vi "Visu acqui 2.vi"() -> ()   [LabVIEW 2022 SP3]
uses:
  Enum/Enum 7.ctl
  Variables globales/Variable glob generale.vi
  Variables globales/Variable globale compteurs.vi
  Variables globales/Variable glob Keller.vi
  Variables globales/Variable glob Pt.vi
  Variables globales/Variable glob Leybold.vi
  Variables globales/Variable glob Edwards.vi
  Variables globales/Variable glob Th.vi
  Variables globales/Variables glob EUROTHERM.vi
  Variables globales/Variable glob alertes pressions.vi
  Variables globales/Variable glob alertes min-max temperatures.vi
  Variables globales/Variable glob alertes ecart temperatures.vi
  Variables globales/Variable glob alertes Keller.vi
  Variables globales/Variable glob alertes Compteurs.vi
  <vilib>/Utility/config.llb/Write Key (String).vi
  <vilib>/Utility/config.llb/NI_LVConfig.lvlib
panel:
  in  "Légende":T1(array[cluster])
  out "Alerte Compteurs":bool
  in  "voir compteurs":bool caption="Valeurs compteurs"
  in  "Unités par":u16(ring) items=["seconde", "minute", "heure"]
  out "Pente":dbl format="%#.2g"
  in  "Capteur":u16(ring) items=["Puissance Reg REG_TABLE", "Mesure Reg REG_TABLE", "Consigne Reg REG_TABLE", "Sécurité Reg REG_TABLE", "Alarme basse Reg REG_TABLE", "Alarme haute RegREG_TABLE"]
  in  "Calcul Pente":bool
  in  "voir alertes":bool caption="Définitions Alertes"
  out "nb capt":i32
  out "Cuve":string
  out "Dossier distant":path
  out "référence en sortie":refnum<vi>
  out "SORTIE VISU":bool
  in  "Tout Y2":bool
  out "commentaire":string
  out "Dossier de sauvegarde":path
  in  "Tout Y1":bool
  in  "Tout OFF":bool
  out "Chemin du fichier local":path
  out "Alerte écart temp":bool caption="Alerte écarts températures"
  in  "Y2 log":bool caption="Y2 lin"
  in  "Y1 log":bool caption="Y1 lin"
  out "Alerte Keller":bool
  out "Alerte min/max temp":bool caption="Alerte min/max températures"
  out "Alerte vide":bool
  in  "grille Y2":bool
  in  "grille Y1":bool
  out "Courbe":cluster{dbl[], dbl[]}[](graph)
  in  "Echelles des Axes":bool=TRUE
  in  "SORTIR VISU":bool
  # "VISUALISATION ACQUISITIONS\ntempératures et pressions EN COURS"
  # "Ce logiciel et les informations qu'il contient, sont la propriété de l’IAS et ne peuvent être diffusés sans l’autorisation de la Station d’étalonnage"
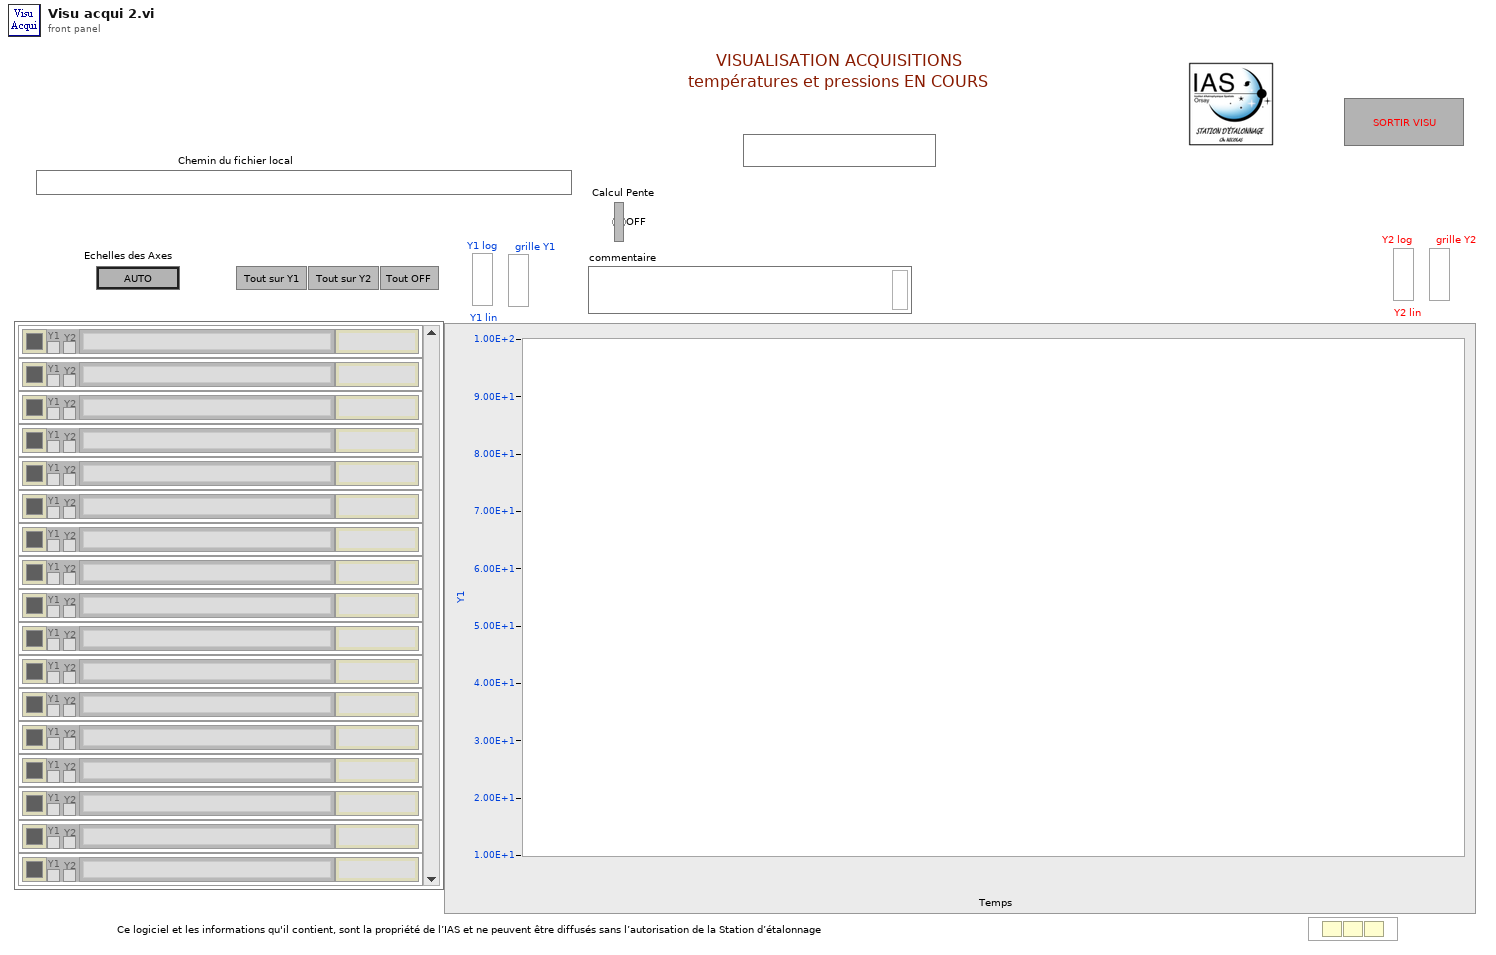
[diagram p1: front panel]
types:
  T1 = cluster{"couleur":u32, "Y1":bool, "nom":string, "donnée":string, "Y2":bool}[]
  T2 = typedef "Enum 7.ctl" = enum16{"init", "choix", "init graph", "visu", "choix 2", "fin"}
  T3 = enum32{"Invalid", "Standard", "Closed", "Hidden", "Minimized", "Maximized"}
  T4 = cluster{"Noms voies select acqui 1COM":string[]}[]
  T5 = cluster{"Nom tache compteurs":refnum<k21>, "Noms des compteurs":string[], "Selection":bool[], "Init compteurs":dbl[], "Noms compteurs selectionnes":string[]}
  T6 = cluster{"Nom tache Pt":refnum<k21>, "Noms des Pt":string[], "Nb Pt":i16, "Selection Pt":bool[], "Nom Pt selectionnees":string[]}[]
  T7 = cluster{"Nom tache Th":refnum<k21>, "Noms des Th":string[], "Nb Th":i16, "Selection Th":bool[], "Nom Th selectionnes":string[]}[]
  T8 = cluster{"couleur":u32, "Y1":bool, "nom":string, "donnée":string, "Y2":bool}
  T9 = cluster{"Alerte temp min/max":bool, "température max":dbl, "température min":dbl, "Défaut min/max temp":bool, "Indices à controler":i16[], "N°":u16}[]
  T10 = cluster{"Indices a controler":i16[], "Defaut":bool, "ecart temp":dbl, "Alerte":bool, ">?":bool, "N°":u16}[]
  T11 = cluster{"Alerte":bool, "valeur alerte":dbl, "Défaut":bool, "Indices à controler":i16[], "N°":u16}[]
  T12 = cluster{"Alerte":bool, "valeur ":dbl, "Défaut":bool, "Indices controler":i16[], "N°":u16}[]
  T13 = cluster{"Alerte Keller":bool, "valeur alerte Keller":dbl, "Défaut Keller":bool, "Indices Keller à controler":i16[], "N°":u16}[]
  T14 = typedef "NI_LVConfig.lvlib/Config Data RefNum.ctl" = refnum<k1>
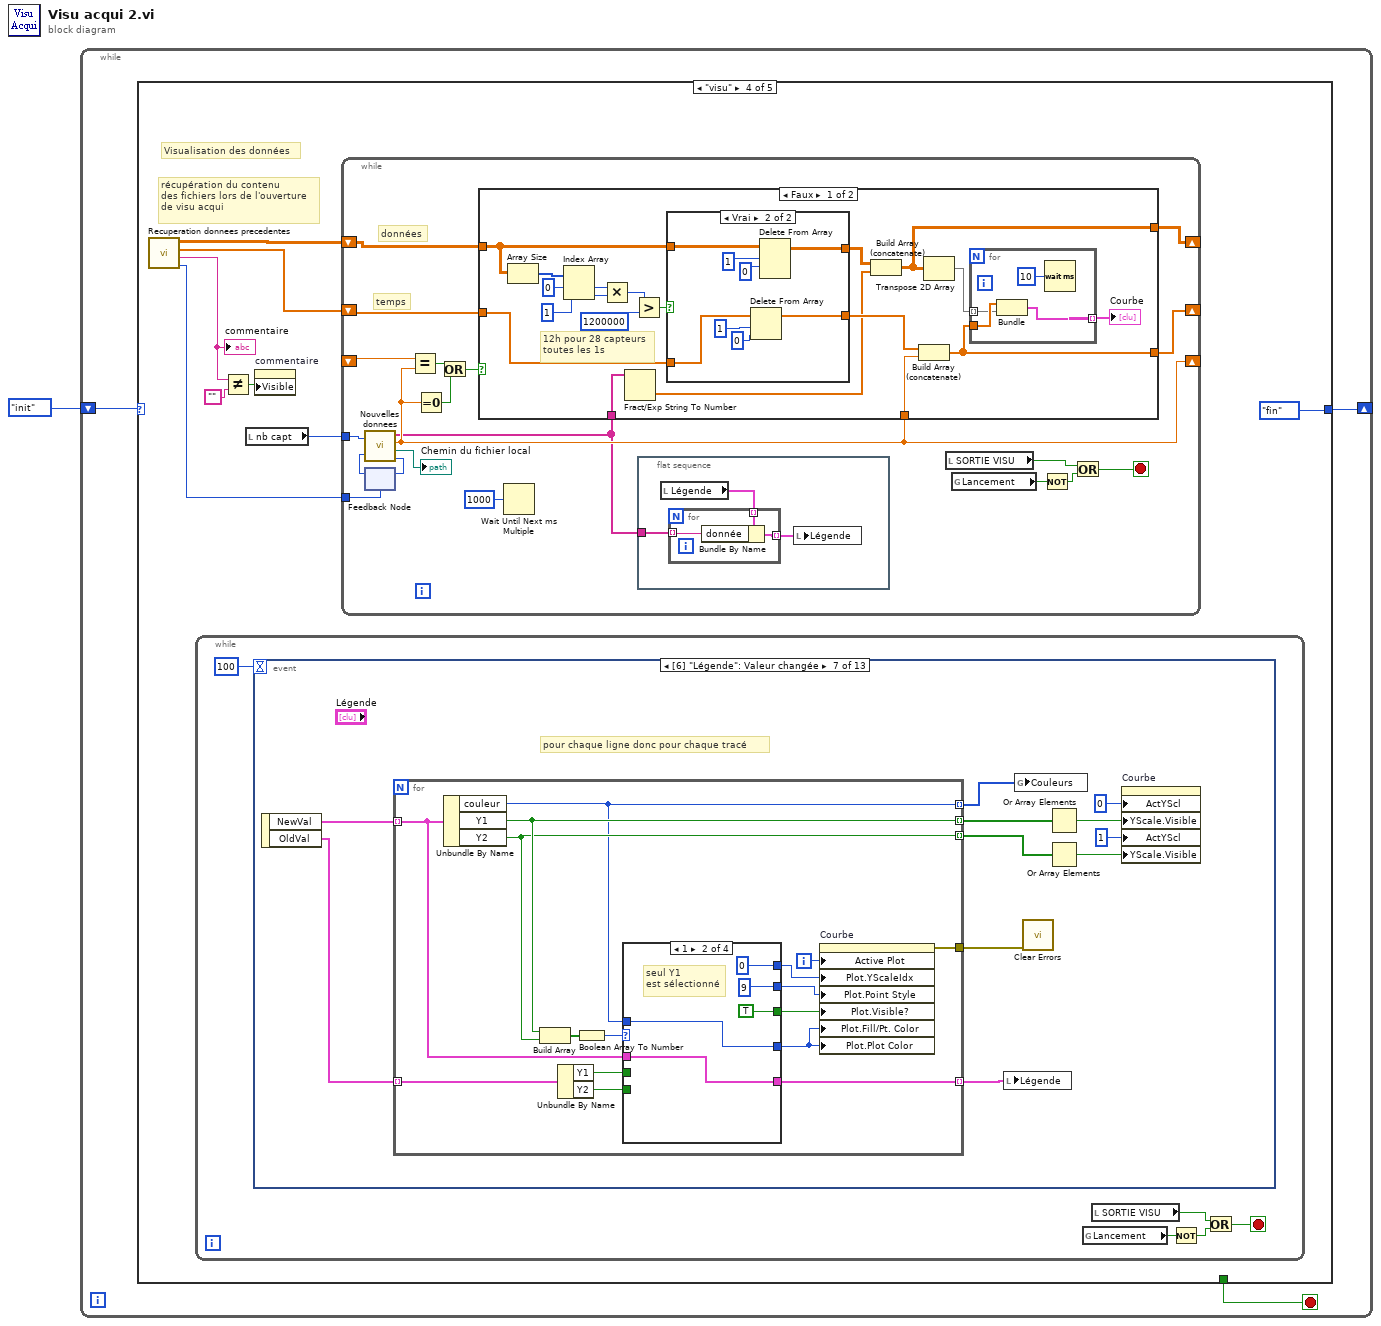
[diagram p0: block diagram]
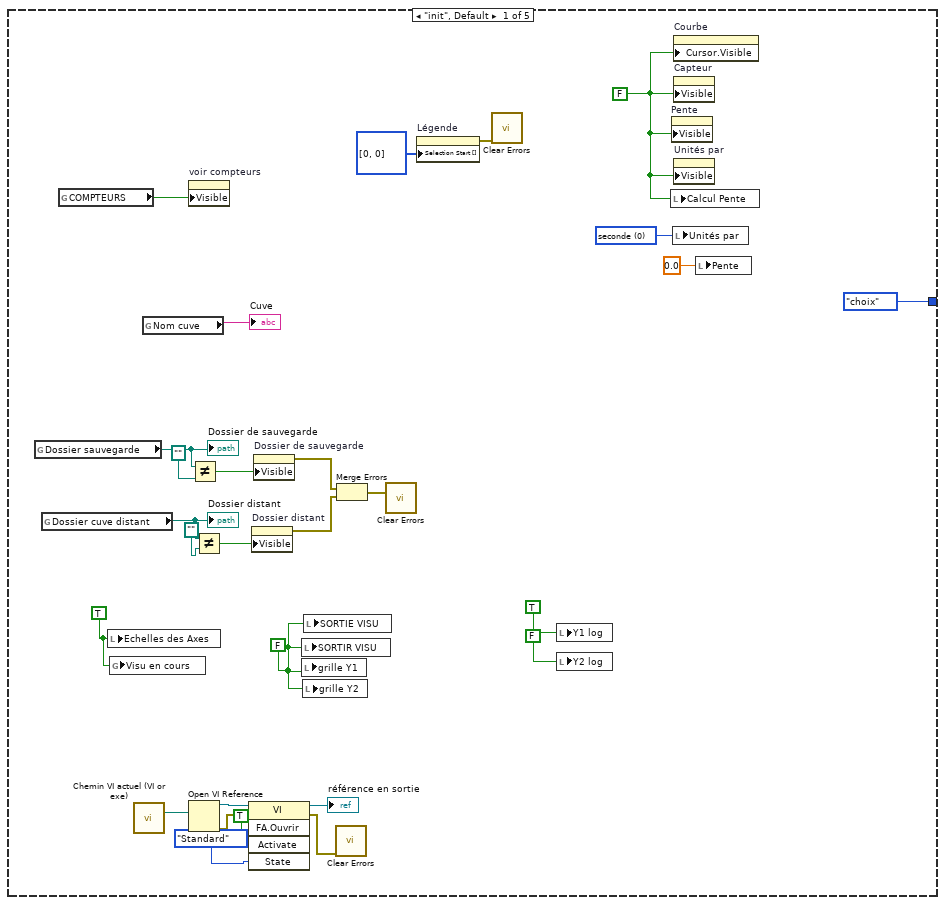
[diagram p2: hidden frame]
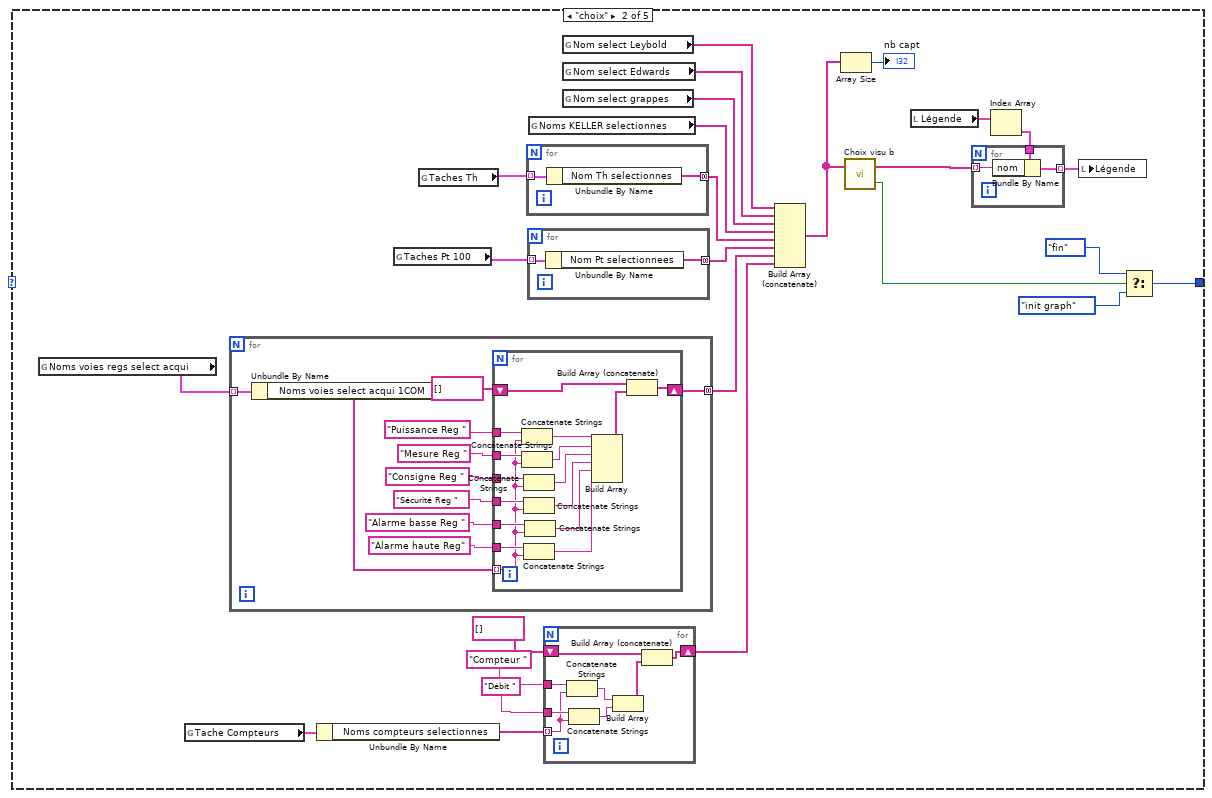
[diagram p3: hidden frame]
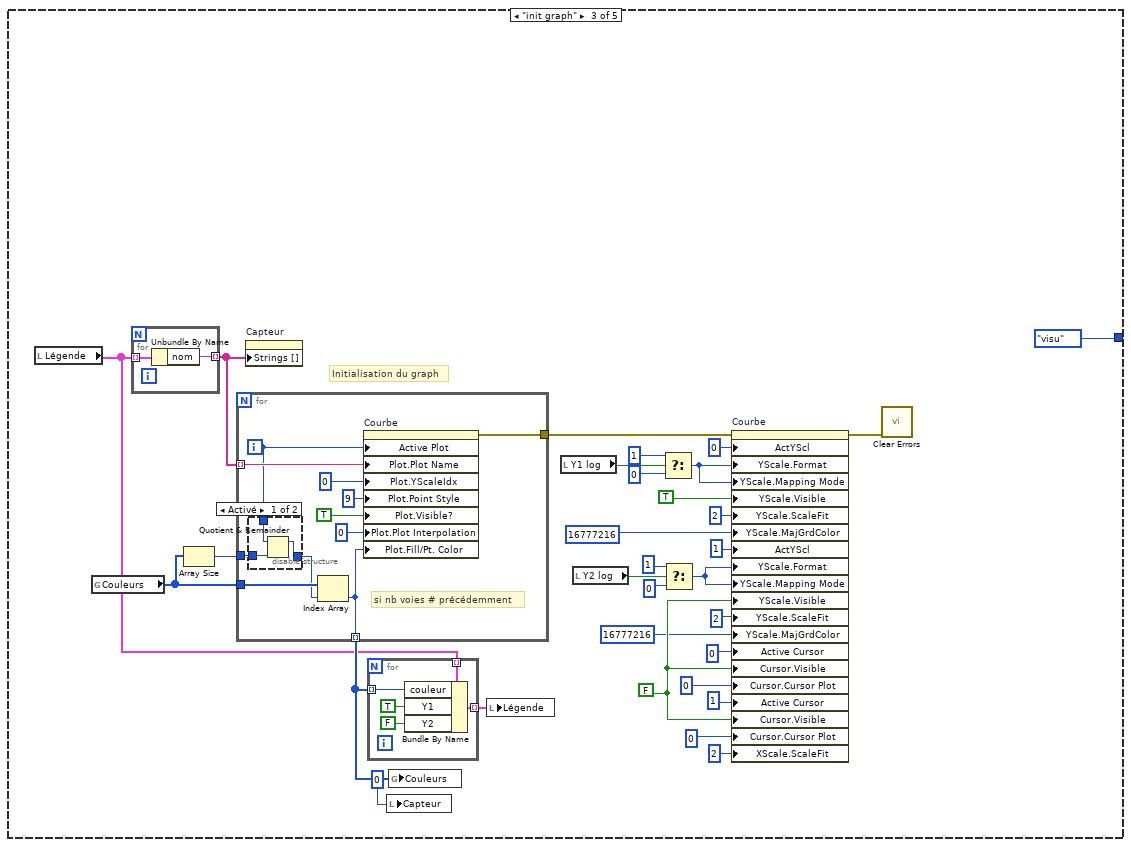
[diagram p4: hidden frame]
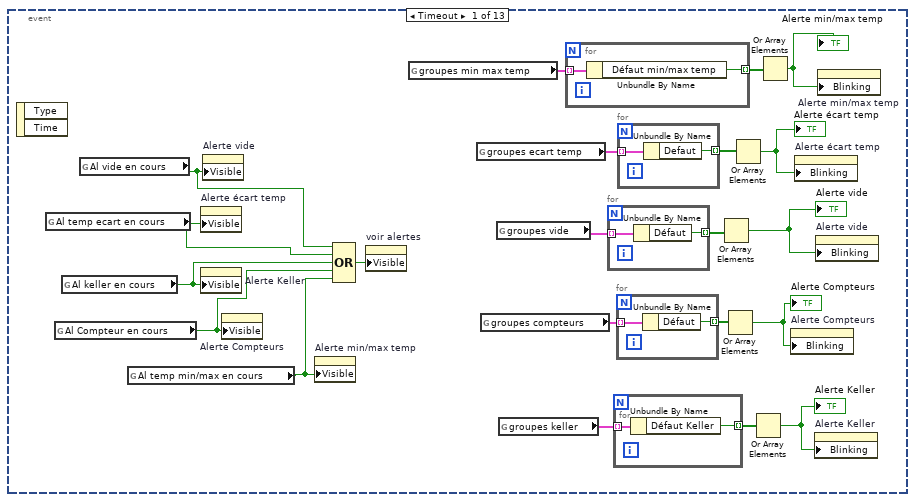
[diagram p6: hidden frame]
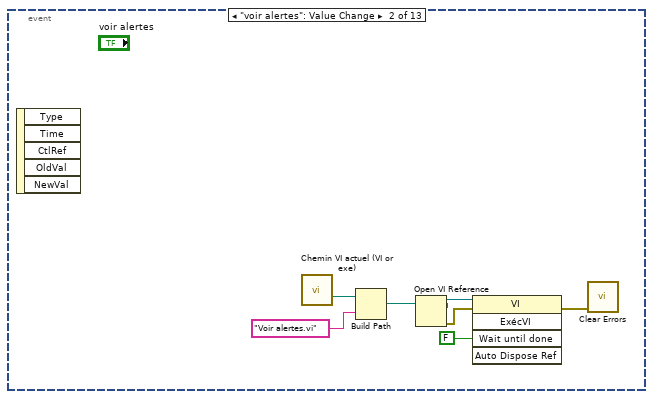
[diagram p7: hidden frame]
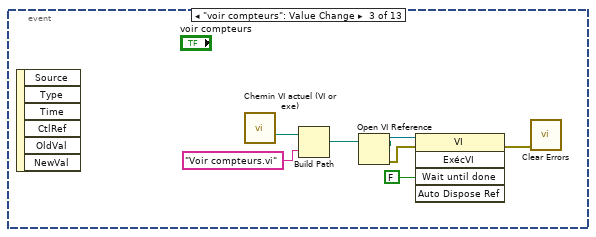
[diagram p8: hidden frame]
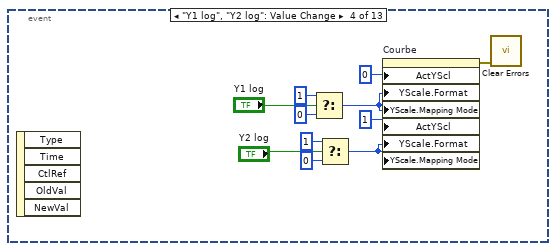
[diagram p9: hidden frame]
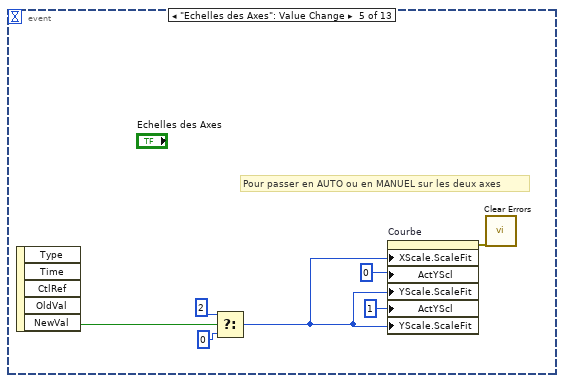
[diagram p10: hidden frame]
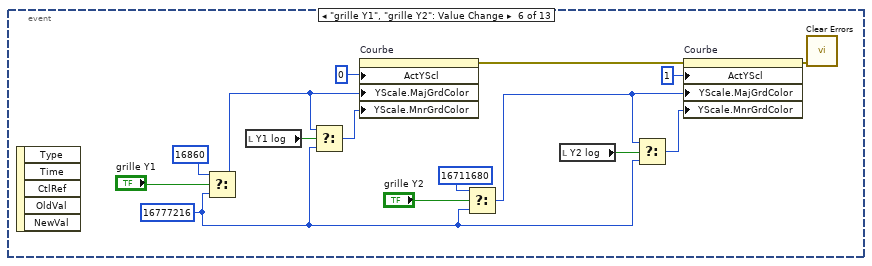
[diagram p11: hidden frame]
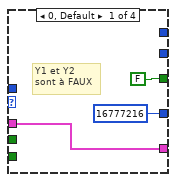
[diagram p12: hidden frame]
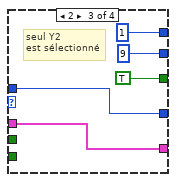
[diagram p13: hidden frame]
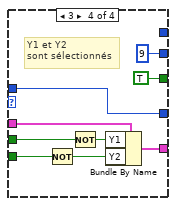
[diagram p14: hidden frame]
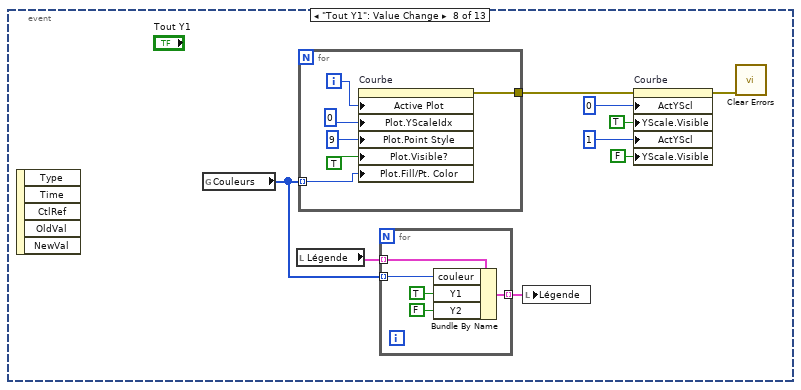
[diagram p15: hidden frame]
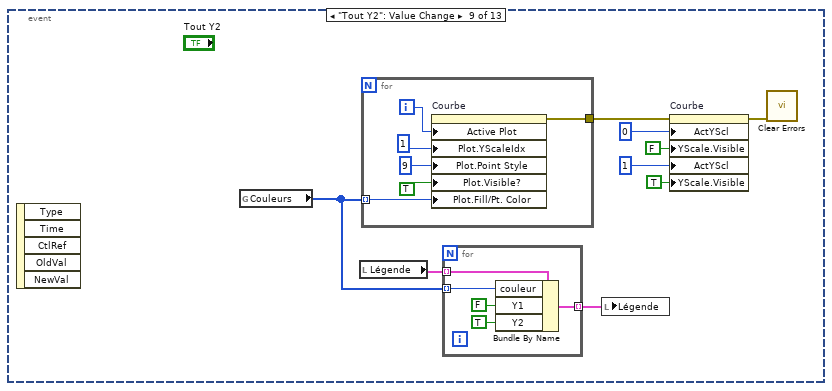
[diagram p16: hidden frame]
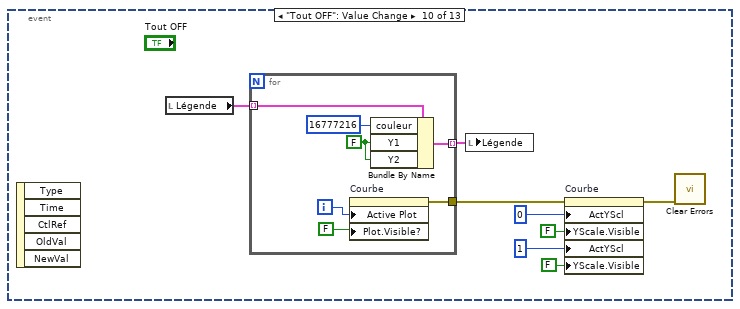
[diagram p17: hidden frame]
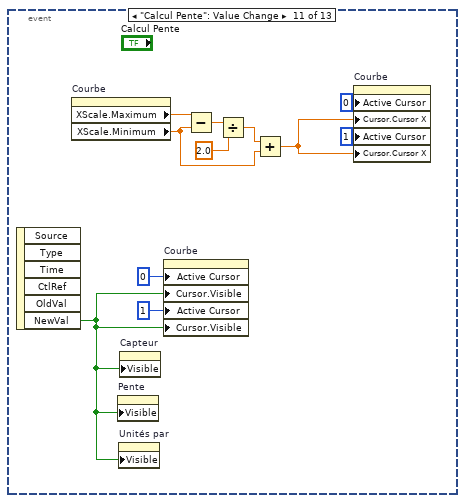
[diagram p18: hidden frame]
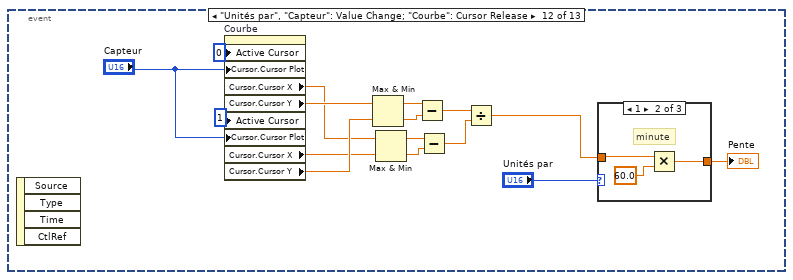
[diagram p19: hidden frame]
diagram:
  n1 = while {
    shift-right: [w3] -> _
    shift-left: Enum_7."init" ("Énum") -> [w4]
    stop <- w2 stop-if-true
    n2 = case shown="\"visu\"" w4 {
      tunnel: [Enum_7."choix" ("Énum") w50 Enum_7."visu" ("Énum") Enum_7."fin" ("Énum") Enum_7."init" ("Énum")] -> w3
      tunnel: [_ _ _ _ TRUE] -> w2
      frame "init", Default {
        w7 = u16 0 items=["seconde", "minute", "heure"] ("Unités par")
        w10 = FALSE
        w31 = TRUE ("Echelles des Axes")
        w32 = FALSE
        n3 = global read "Variable glob generale.vi" "Dossier sauvegarde"() -> (w30:path)
        "Dossier de sauvegarde" <- w30
        n4 = global read "Variable glob generale.vi" "Dossier cuve distant"() -> (w27:path)
        "Dossier distant" <- w27
        n5 = global read "Variable globale compteurs.vi" "COMPTEURS"() -> (w8:bool)
        n6 = local write "Echelles des Axes"(w31) -> ()
        n7 = global write "Variable glob generale.vi" "Visu en cours"(w31) -> ()
        n8 = call "Chemin VI actuel (VI or exe).vi"() -> ("Full Path to VI or executable"=w13:path)  [unwired: 14 in, 1 out]
        n9 = global read "Variable glob generale.vi" "Nom cuve"() -> (→"Cuve":string)
        n10 = property on="voir compteurs" class="Bool"("Visible"=w8) -> ()  [unwired: 2 in, 2 out]
        n11 = Open VI Reference(vi path=w13) -> (vi reference=w17:refnum<vi>, error out=w15:errorcluster)  [unwired: 5 in]
        n12 = Not Equal?(x=w30, y=path "") -> (x != y?=w28:bool)
        n13 = Not Equal?(x=w27, y=path "") -> (x != y?=w25:bool)
        n14 = invoke class="VI" method="FA.Ouvrir"(reference=w17, error in=w15, "Activate"=TRUE ("Activer ?"), "State"=T3."Standard" ("État")) -> (reference out=→"référence en sortie":refnum<vi>, error out=w14:errorcluster)  [unwired: 1 in, 3 out]
        n15 = property on="Dossier distant" class="Chm"("Visible"=w25) -> (error out=w22:errorcluster)  [unwired: 2 in, 1 out]
        n16 = property on="Dossier de sauvegarde" class="Chm"("Visible"=w28) -> (error out=w23:errorcluster)  [unwired: 2 in, 1 out]
        n17 = local write "SORTIR VISU"(w32) -> ()
        n18 = local write "grille Y1"(w32) -> ()
        n19 = local write "grille Y2"(w32) -> ()
        n20 = local write "SORTIE VISU"(w32) -> ()
        n21 = call <vilib>:"Clear Errors.vi"("error in (no error)"=w14) -> ()  [unwired: 5 in, 2 out]
        n22 = Merge Errors(w23, w22) -> (w24:errorcluster)
        n23 = call <vilib>:"Clear Errors.vi"("error in (no error)"=w24) -> ()  [unwired: 5 in, 2 out]
        n24 = property on="Légende" class="Tabl (strict)"("Selection Start []"=u32[] [0, 0] ("Début de sélection []")) -> (error out=w5:errorcluster)  [unwired: 2 in, 1 out]
        n25 = call <vilib>:"Clear Errors.vi"("error in (no error)"=w5) -> ()  [unwired: 5 in, 2 out]
        n26 = local write "Y1 log"(TRUE ("Y1 log")) -> ()
        n27 = local write "Y2 log"(FALSE ("Y2 log")) -> ()
        n28 = local write "Calcul Pente"(w10) -> ()
        n29 = property on="Pente" class="NumNb (strict)"("Visible"=w10) -> ()  [unwired: 2 in, 2 out]
        n30 = local write "Unités par"(w7) -> ()
        n31 = property on="Courbe" class="GraphXY (strict)"("Cursor.Visible"=w10) -> ()  [unwired: 2 in, 2 out]
        n32 = property on="Capteur" class="MDér (strict)"("Visible"=w10) -> ()  [unwired: 2 in, 2 out]
        n33 = property on="Unités par" class="MDér (strict)"("Visible"=w10) -> ()  [unwired: 2 in, 2 out]
        n34 = local write "Pente"(0.0 ("Pente")) -> ()
      }
      frame "choix" {
        n35 = global read "Variables glob EUROTHERM.vi" "Noms voies regs select acqui"() -> (w44:T4)
        n36 = global read "Variable globale compteurs.vi" "Tache Compteurs"() -> (w42:T5)
        n37 = for {
          tunnel: w44 -> [w79] mode=indexing
          tunnel: [w70] -> w43 mode=concatenating
          n38 = Unbundle By Name(w79) -> ("Noms voies select acqui 1COM"=w71:string[])
          n39 = for {
            tunnel: w71 -> [w89] mode=indexing
            tunnel: "Puissance Reg " -> [w95]
            tunnel: "Mesure Reg " -> [w94]
            tunnel: "Consigne Reg " -> [w93]
            tunnel: "Sécurité Reg " -> [w92]
            tunnel: "Alarme basse Reg " -> [w91]
            tunnel: "Alarme haute Reg" -> [w90]
            shift-right: [w80] -> w70
            shift-left: string[] [] -> [w81]
            n40 = Concatenate Strings(w95, w89) -> (w88:string)
            n41 = Concatenate Strings(w94, w89) -> (w87:string)
            n42 = Concatenate Strings(w93, w89) -> (w86:string)
            n43 = Concatenate Strings(w92, w89) -> (w85:string)
            n44 = Concatenate Strings(w90, w89) -> (w83:string)
            n45 = Concatenate Strings(w91, w89) -> (w84:string)
            n46 = Build Array(w88, w87, w86, w85, w84, w83) -> (w82:string[])
            n47 = Build Array (concatenate)(w81, w82) -> (w80:string[])
          }
        }
        n48 = Unbundle By Name(w42) -> ("Noms compteurs selectionnes"=w41:string[])
        n49 = global read "Variable glob Pt.vi" "Taches Pt 100"() -> (w48:T6)
        n50 = global read "Variable glob Th.vi" "Taches Th"() -> (w46:T7)
        n51 = for {
          tunnel: w46 -> [w97] mode=indexing
          tunnel: [w96] -> w45 mode=concatenating
          n52 = Unbundle By Name(w97) -> ("Nom Th selectionnes"=w96:string[])
        }
        n53 = for {
          tunnel: w48 -> [w99] mode=indexing
          tunnel: [w98] -> w47 mode=concatenating
          n54 = Unbundle By Name(w99) -> ("Nom Pt selectionnees"=w98:string[])
        }
        n55 = global read "Variable glob Keller.vi" "Noms KELLER selectionnes"() -> (w56:string[])
        n56 = for {
          tunnel: w41 -> [w67] mode=indexing
          tunnel: "Compteur " -> [w69]
          tunnel: "Débit " -> [w68]
          shift-right: [w63] -> w37
          shift-left: string[] [] -> [w64]
          n57 = Concatenate Strings(w69, w67) -> (w66:string)
          n58 = Concatenate Strings(w68, w67) -> (w65:string)
          n59 = Build Array(w66, w65) -> (w62:string[])
          n60 = Build Array (concatenate)(w64, w62) -> (w63:string[])
        }
        n61 = global read "Variable glob Leybold.vi" "Nom select Leybold"() -> (w57:string[])
        n62 = global read "Variable glob Edwards.vi" "Nom select Edwards"() -> (w58:string[])
        n63 = global read "Variable glob Edwards.vi" "Nom select grappes"() -> (w49:string[])
        n64 = Build Array (concatenate)(w57, w58, w49, w56, w45, w47, w43, w37) -> (w54:string[])
        n65 = Array Size(array=w54) -> (size(s)=→"nb capt":i32)
        n66 = call "Choix visu b.vi"("Noms"=w54) -> ("annulé"=w53:bool, "Noms 2"=w36:string[])  [unwired: 1 in]
        n67 = local read "Légende"() -> (w33:T1)
        n68 = Index Array(array=w33) -> (element=w34:T8)  [unwired: 1 in]
        n69 = for {
          tunnel: [w61] -> w35 mode=indexing
          tunnel: w36 -> [w60] mode=indexing
          tunnel: w34 -> [w59]
          n70 = Bundle By Name(cluster=w59, "nom"=w60) -> (w61:T8)
        }
        n71 = local write "Légende"(w35) -> ()
        n72 = Select(t=Enum_7."fin" ("Énum"), s=w53, f=Enum_7."init graph" ("Énum")) -> (s? t:f=w50:T2)
      }
      frame "init graph" {
        w112 = FALSE ("Échelle des Y.Visible")
        # "Initialisation du graph"
        n73 = local read "Légende"() -> (w100:T1)
        n74 = global read "Variable glob generale.vi" "Couleurs"() -> (w130:u32[])
        n75 = for {
          tunnel: w100 -> [w137] mode=indexing
          tunnel: [w136] -> w103 mode=indexing
          n76 = Unbundle By Name(w137) -> ("nom"=w136:string)
        }
        n77 = Array Size(array=w130) -> (size(s)=w129:i32)
        n78 = for {
          tunnel: w103 -> [w148] mode=indexing
          tunnel: [w142] -> w102 mode=indexing
          tunnel: w130 -> [w143]
          tunnel: w129 -> [w140]
          tunnel: [w139] -> w127
          i -> [w138]
          # "si nb voies # précédemment"
          n79 = disable-structure shown="Activé" {
            disable-tunnel: [w151 w152] -> w141
            disable-tunnel: w140 -> [w150 _]
            disable-tunnel: w138 -> [w149 w152]
            frame Enabled {
              n80 = Quotient & Remainder(x=w149, y=w150) -> (x-y*floor(x/y)=w151:i32)  [unwired: 1 out]
            }
            frame Disabled {
            }
          }
          n81 = Index Array(array=w143, index=w141) -> (element=w142:u32)
          n82 = property on="Courbe" class="GraphXY (strict)"("Active Plot"=w138, "Plot.Plot Name"=w148, "Plot.YScaleIdx"=u32 0 ("Tracé.Indice d'échelle des Y"), "Plot.Point Style"=u8 9 ("Tracé.Style de point"), "Plot.Visible?"=TRUE, "Plot.Plot Interpolation"=u32 0 ("Tracé.Indice d'échelle des Y"), "Plot.Fill/Pt. Color"=w142) -> (error out=w139:errorcluster)  [unwired: 2 in, 1 out]
        }
        n83 = property on="Capteur" class="MDér (strict)"("Strings []"=w103) -> ()  [unwired: 2 in, 2 out]
        n84 = for {
          tunnel: w100 -> [w135] mode=indexing
          tunnel: w102 -> [w134] mode=indexing
          tunnel: [w133] -> w101 mode=indexing
          n85 = Bundle By Name(cluster=w135, "couleur"=w134, "Y1"=TRUE, "Y2"=FALSE) -> (w133:T8)
        }
        n86 = local write "Capteur"(u16 0) -> ()
        n87 = global write "Variable glob generale.vi" "Couleurs"(w102) -> ()
        n88 = local write "Légende"(w101) -> ()
        n89 = local read "Y1 log"() -> (w119:bool)
        n90 = local read "Y2 log"() -> (w118:bool)
        n91 = Select(t=u8 1 ("cas vrai"), s=w119, f=u8 0 ("cas faux")) -> (s? t:f=w120:u8)
        n92 = Select(t=u8 1 ("cas vrai"), s=w118, f=u8 0 ("cas faux")) -> (s? t:f=w116:u8)
        n93 = property on="Courbe" class="GraphXY (strict)"(error in=w127, "ActYScl"=0 ("Échelle active des Y"), "YScale.Format"=w120, "YScale.Mapping Mode"=w120, "YScale.Visible"=TRUE ("Échelle des Y.Visible"), "YScale.ScaleFit"=u8 2 ("Échelle des X.Ajuster l'échelle"), "YScale.MajGrdColor"=u32 16777216 ("cas faux"), "ActYScl"=1 ("Échelle active des Y"), "YScale.Format"=w116, "YScale.Mapping Mode"=w116, "YScale.Visible"=w112, "YScale.ScaleFit"=u8 2 ("Échelle des X.Ajuster l'échelle"), "YScale.MajGrdColor"=u32 16777216 ("cas faux"), "Active Cursor"=u32 0 ("Curseur actif"), "Cursor.Visible"=w112, "Cursor.Cursor Plot"=0 ("Curseur.Tracé du curseur"), "Active Cursor"=u32 1 ("Curseur actif"), "Cursor.Visible"=w112, "Cursor.Cursor Plot"=0 ("Curseur.Tracé du curseur"), "XScale.ScaleFit"=u8 2 ("Échelle des X.Ajuster l'échelle")) -> (error out=w126:errorcluster)  [unwired: 1 in, 1 out]
        n94 = call <vilib>:"Clear Errors.vi"("error in (no error)"=w126) -> ()  [unwired: 5 in, 2 out]
      }
      frame "visu" {
        # "récupération du contenu\ndes fichiers lors de l'ouverture\nde visu acqui"
        # "Visualisation des données"
        n95 = call "Recuperation donnees precedentes.vi"() -> ("Données"=w160:dbl[][], "Temps"=w159:dbl[], "commentaire"=w158:string, "offset (en octets)"=w155:i64)  [unwired: 2 in]
        "commentaire" <- w158
        n96 = while {
          stop <- w164 stop-if-true
          n97 = event shown="[6] \"Légende\": Valeur changée" {
            selector: _ -> [_ _ _ _ _ _ _ _ _ _ _ _ _]
            dyn-events: _ -> [_ _ _ _ _ _ _ _ _ _ _ _ _]
            timeout: 100 -> [_ _ _ _ _ _ _ _ _ _ _ _ _]
            event Timeout {
              n98 = event-data() -> ()  [unwired: 1 in, 2 out]
              n99 = global read "Variable glob alertes ecart temperatures.vi" "Al temp ecart en cours"() -> (w184:bool)
              n100 = global read "Variable glob alertes Compteurs.vi" "Al Compteur en cours"() -> (w181:bool)
              n101 = global read "Variable glob alertes Keller.vi" "Al keller en cours"() -> (w183:bool)
              n102 = global read "Variable glob alertes pressions.vi" "Al vide en cours"() -> (w185:bool)
              n103 = global read "Variable glob alertes min-max temperatures.vi" "Al temp min/max en cours"() -> (w182:bool)
              n104 = property on="Alerte écart temp" class="Bool (strict)"("Visible"=w184) -> ()  [unwired: 2 in, 2 out]
              n105 = property on="Alerte Keller" class="Bool (strict)"("Visible"=w183) -> ()  [unwired: 2 in, 2 out]
              n106 = property on="Alerte vide" class="Bool (strict)"("Visible"=w185) -> ()  [unwired: 2 in, 2 out]
              n107 = property on="Alerte Compteurs" class="Bool (strict)"("Visible"=w181) -> ()  [unwired: 2 in, 2 out]
              n108 = property on="Alerte min/max temp" class="Bool (strict)"("Visible"=w182) -> ()  [unwired: 2 in, 2 out]
              n109 = Compound Arithmetic op=OR(w185, w184, w183, w181, w182) -> (w186:bool)
              n110 = property on="voir alertes" class="Bool"("Visible"=w186) -> ()  [unwired: 2 in, 2 out]
              n111 = global read "Variable glob alertes min-max temperatures.vi" "groupes min max temp"() -> (w177:T9)
              n112 = global read "Variable glob alertes ecart temperatures.vi" "groupes ecart temp"() -> (w180:T10)
              n113 = global read "Variable glob alertes Compteurs.vi" "groupes compteurs"() -> (w168:T11)
              n114 = global read "Variable glob alertes pressions.vi" "groupes vide"() -> (w171:T12)
              n115 = global read "Variable glob alertes Keller.vi" "groupes keller"() -> (w174:T13)
              n116 = for {
                tunnel: w177 -> [w194] mode=indexing
                tunnel: [w193] -> w176 mode=indexing
                n117 = Unbundle By Name(w194) -> ("Défaut min/max temp"=w193:bool)
              }
              n118 = for {
                tunnel: w171 -> [w190] mode=indexing
                tunnel: [w189] -> w170 mode=indexing
                n119 = Unbundle By Name(w190) -> ("Défaut"=w189:bool)
              }
              n120 = for {
                tunnel: w174 -> [w192] mode=indexing
                tunnel: [w191] -> w173 mode=indexing
                n121 = Unbundle By Name(w192) -> ("Défaut Keller"=w191:bool)
              }
              n122 = for {
                tunnel: w168 -> [w188] mode=indexing
                tunnel: [w187] -> w167 mode=indexing
                n123 = Unbundle By Name(w188) -> ("Défaut"=w187:bool)
              }
              n124 = for {
                tunnel: w180 -> [w196] mode=indexing
                tunnel: [w195] -> w179 mode=indexing
                n125 = Unbundle By Name(w196) -> ("Defaut"=w195:bool)
              }
              n126 = Or Array Elements(Boolean array=w170) -> (logical OR=w169:bool)
              "Alerte vide" <- w169
              n127 = Or Array Elements(Boolean array=w167) -> (logical OR=w166:bool)
              "Alerte Compteurs" <- w166
              n128 = Or Array Elements(Boolean array=w179) -> (logical OR=w178:bool)
              "Alerte écart temp" <- w178
              n129 = Or Array Elements(Boolean array=w173) -> (logical OR=w172:bool)
              "Alerte Keller" <- w172
              n130 = Or Array Elements(Boolean array=w176) -> (logical OR=w175:bool)
              "Alerte min/max temp" <- w175
              n131 = property on="Alerte Compteurs" class="Bool (strict)"("Blinking"=w166) -> ()  [unwired: 2 in, 2 out]
              n132 = property on="Alerte écart temp" class="Bool (strict)"("Blinking"=w178) -> ()  [unwired: 2 in, 2 out]
              n133 = property on="Alerte Keller" class="Bool (strict)"("Blinking"=w172) -> ()  [unwired: 2 in, 2 out]
              n134 = property on="Alerte vide" class="Bool (strict)"("Blinking"=w169) -> ()  [unwired: 2 in, 2 out]
              n135 = property on="Alerte min/max temp" class="Bool (strict)"("Blinking"=w175) -> ()  [unwired: 2 in, 2 out]
            }
            event "voir alertes": Value Change {
              n136 = event-data() -> ()  [unwired: 1 in, 5 out]
              n137 = call "Chemin VI actuel (VI or exe).vi"() -> ("VI or executable installation directory"=w197:path)  [unwired: 14 in, 1 out]
              n138 = Build Path(base path=w197, name or relative path="Voir alertes.vi" ("nom ou chemin relatif")) -> (appended path=w202:path)
              n139 = Open VI Reference(vi path=w202) -> (vi reference=w200:refnum<vi>, error out=w199:errorcluster)  [unwired: 5 in]
              n140 = invoke class="VI" method="ExécVI"(reference=w200, error in=w199, "Wait until done"=FALSE ("Attendre la fin")) -> (error out=w198:errorcluster)  [unwired: 2 in, 4 out]
              n141 = call <vilib>:"Clear Errors.vi"("error in (no error)"=w198) -> ()  [unwired: 5 in, 2 out]
            }
            event "voir compteurs": Value Change {
              n142 = event-data() -> ()  [unwired: 1 in, 6 out]
              n143 = call "Chemin VI actuel (VI or exe).vi"() -> ("VI or executable installation directory"=w206:path)  [unwired: 14 in, 1 out]
              n144 = Build Path(base path=w206, name or relative path="Voir compteurs.vi" ("nom ou chemin relatif")) -> (appended path=w210:path)
              n145 = Open VI Reference(vi path=w210) -> (vi reference=w209:refnum<vi>, error out=w208:errorcluster)  [unwired: 5 in]
              n146 = invoke class="VI" method="ExécVI"(reference=w209, error in=w208, "Wait until done"=FALSE ("Attendre la fin")) -> (error out=w207:errorcluster)  [unwired: 2 in, 4 out]
              n147 = call <vilib>:"Clear Errors.vi"("error in (no error)"=w207) -> ()  [unwired: 5 in, 2 out]
            }
            event "Y1 log", "Y2 log": Value Change {
              n148 = event-data() -> ()  [unwired: 1 in, 5 out]
              n149 = Select(t=i8 1 ("cas vrai"), s="Y1 log", f=i8 0 ("cas faux")) -> (s? t:f=w217:i8)
              n150 = Select(t=i8 1 ("cas vrai"), s="Y2 log", f=i8 0 ("cas faux")) -> (s? t:f=w220:i8)
              n151 = property on="Courbe" class="GraphXY (strict)"("ActYScl"=0 ("Échelle active des Y"), "YScale.Format"=w217, "YScale.Mapping Mode"=w217, "ActYScl"=1 ("Échelle active des Y"), "YScale.Format"=w220, "YScale.Mapping Mode"=w220) -> (error out=w211:errorcluster)  [unwired: 2 in, 1 out]
              n152 = call <vilib>:"Clear Errors.vi"("error in (no error)"=w211) -> ()  [unwired: 5 in, 2 out]
            }
            event "Echelles des Axes": Value Change {
              # "Pour passer en AUTO ou en MANUEL sur les deux axes"
              n153 = event-data() -> ("NewVal"=w226:bool)  [unwired: 1 in, 4 out]
              n154 = Select(t=u8 2 ("cas vrai"), s=w226, f=u8 0 ("Échelle des X.Ajuster l'échelle")) -> (s? t:f=w224:u8)
              n155 = property on="Courbe" class="GraphXY (strict)"("XScale.ScaleFit"=w224, "ActYScl"=0, "YScale.ScaleFit"=w224, "ActYScl"=1, "YScale.ScaleFit"=w224) -> (error out=w222:errorcluster)  [unwired: 2 in, 1 out]
              n156 = call <vilib>:"Clear Errors.vi"("error in (no error)"=w222) -> ()  [unwired: 5 in, 2 out]
            }
            event "grille Y1", "grille Y2": Value Change {
              w229 = 16777216 ("cas faux")
              n157 = event-data() -> ()  [unwired: 1 in, 5 out]
              n158 = Select(t=16860 ("cas vrai"), s="grille Y1", f=w229) -> (s? t:f=w233:i32)
              n159 = local read "Y1 log"() -> (w235:bool)
              n160 = Select(t=w233, s=w235, f=w229) -> (s? t:f=w234:i32)
              n161 = property on="Courbe" class="GraphXY (strict)"("ActYScl"=0 ("Échelle active des Y"), "YScale.MajGrdColor"=w233, "YScale.MnrGrdColor"=w234) -> (error out=w242:errorcluster)  [unwired: 2 in, 1 out]
              n162 = Select(t=16711680 ("cas vrai"), s="grille Y2", f=w229) -> (s? t:f=w231:i32)
              n163 = local read "Y2 log"() -> (w232:bool)
              n164 = Select(t=w231, s=w232, f=w229) -> (s? t:f=w230:i32)
              n165 = property on="Courbe" class="GraphXY (strict)"(error in=w242, "ActYScl"=1 ("Échelle active des Y"), "YScale.MajGrdColor"=w231, "YScale.MnrGrdColor"=w230) -> (error out=w236:errorcluster)  [unwired: 1 in, 1 out]
              n166 = call <vilib>:"Clear Errors.vi"("error in (no error)"=w236) -> ()  [unwired: 5 in, 2 out]
            }
            event "Légende": Value Change {
              # "pour chaque ligne donc pour chaque tracé"
              n167 = event-data() -> ("NewVal"=w248:T1, "OldVal"=w245:T1)  [unwired: 1 in]
              n168 = for {
                tunnel: [w269] -> w254
                tunnel: w248 -> [w256] mode=indexing
                tunnel: [w255] -> w253 mode=indexing
                tunnel: [w268] -> w247 mode=indexing
                tunnel: [w267] -> w246 mode=indexing
                tunnel: w245 -> [w259] mode=indexing
                tunnel: [w258] -> w244 mode=indexing
                i -> [w270]
                n169 = Unbundle By Name(w256) -> ("couleur"=w255:u32, "Y1"=w268:bool, "Y2"=w267:bool)
                n170 = Build Array(w268, w267) -> (w266:bool[])
                n171 = Unbundle By Name(w259) -> ("Y1"=w260:bool, "Y2"=w257:bool)
                n172 = Boolean Array To Number(Boolean array=w266) -> (number=w265:u32)
                n173 = case shown="1" w265 {
                  tunnel: [u32 16777216 ("nouvel élément/sous-tableau") w274 w279 w285] -> w264
                  tunnel: [_ i8 0 ("cas faux") i8 1 ("cas vrai") _] -> w261
                  tunnel: [_ i8 9 ("cas faux") i8 9 ("cas vrai") i8 9 ("cas vrai")] -> w262
                  tunnel: [FALSE TRUE TRUE TRUE] -> w263
                  tunnel: w260 -> [_ _ _ w287]
                  tunnel: [w271 w275 w280 w290] -> w258
                  tunnel: w257 -> [_ _ _ w289]
                  tunnel: w256 -> [w271 w275 w280 w284]
                  tunnel: w255 -> [_ w274 w279 w285]
                  frame 0, Default {
                    # "Y1 et Y2 \nsont à FAUX"
                  }
                  frame 1 {
                    # "seul Y1 \nest sélectionné"
                  }
                  frame 2 {
                    # "seul Y2 \nest sélectionné"
                  }
                  frame 3 {
                    # "Y1 et Y2 \nsont sélectionnés"
                    n174 = Not(x=w289) -> (.not. x?=w288:bool)
                    n175 = Not(x=w287) -> (.not. x?=w286:bool)
                    n176 = Bundle By Name(cluster=w284, "Y1"=w286, "Y2"=w288) -> (w290:T8)
                  }
                }
                n177 = property on="Courbe" class="GraphXY (strict)"("Active Plot"=w270, "Plot.YScaleIdx"=w261, "Plot.Point Style"=w262, "Plot.Visible?"=w263, "Plot.Fill/Pt. Color"=w264, "Plot.Plot Color"=w264) -> (error out=w269:errorcluster)  [unwired: 2 in, 1 out]
              }
              n178 = local write "Légende"(w244) -> ()
              n179 = global write "Variable glob generale.vi" "Couleurs"(w253) -> ()
              n180 = call <vilib>:"Clear Errors.vi"("error in (no error)"=w254) -> ()  [unwired: 5 in, 2 out]
              n181 = Or Array Elements(Boolean array=w247) -> (logical OR=w252:bool)
              n182 = Or Array Elements(Boolean array=w246) -> (logical OR=w251:bool)
              n183 = property on="Courbe" class="GraphXY (strict)"("ActYScl"=0 ("Échelle active des Y"), "YScale.Visible"=w252, "ActYScl"=1 ("Échelle active des Y"), "YScale.Visible"=w251) -> ()  [unwired: 2 in, 2 out]
            }
            event "Tout Y1": Value Change {
              n184 = event-data() -> ()  [unwired: 1 in, 5 out]
              n185 = global read "Variable glob generale.vi" "Couleurs"() -> (w294:u32[])
              n186 = local read "Légende"() -> (w295:T1)
              n187 = for {
                tunnel: w294 -> [w308] mode=indexing
                tunnel: [w307] -> w297
                i -> [w309]
                n188 = property on="Courbe" class="GraphXY (strict)"("Active Plot"=w309, "Plot.YScaleIdx"=i8 0 ("cas faux"), "Plot.Point Style"=i8 9 ("cas faux"), "Plot.Visible?"=TRUE, "Plot.Fill/Pt. Color"=w308) -> (error out=w307:errorcluster)  [unwired: 2 in, 1 out]
              }
              n189 = for {
                tunnel: w295 -> [w306] mode=indexing
                tunnel: w294 -> [w305] mode=indexing
                tunnel: [w304] -> w293 mode=indexing
                n190 = Bundle By Name(cluster=w306, "couleur"=w305, "Y1"=TRUE, "Y2"=FALSE) -> (w304:T8)
              }
              n191 = local write "Légende"(w293) -> ()
              n192 = property on="Courbe" class="GraphXY (strict)"(error in=w297, "ActYScl"=0 ("Échelle active des Y"), "YScale.Visible"=TRUE ("Échelle des Y.Visible"), "ActYScl"=1 ("Échelle active des Y"), "YScale.Visible"=FALSE ("Échelle des Y.Visible")) -> (error out=w296:errorcluster)  [unwired: 1 in, 1 out]
              n193 = call <vilib>:"Clear Errors.vi"("error in (no error)"=w296) -> ()  [unwired: 5 in, 2 out]
            }
            event "Tout Y2": Value Change {
              n194 = event-data() -> ()  [unwired: 1 in, 5 out]
              n195 = global read "Variable glob generale.vi" "Couleurs"() -> (w313:u32[])
              n196 = local read "Légende"() -> (w315:T1)
              n197 = for {
                tunnel: w313 -> [w328] mode=indexing
                tunnel: [w327] -> w317
                i -> [w329]
                n198 = property on="Courbe" class="GraphXY (strict)"("Active Plot"=w329, "Plot.YScaleIdx"=i8 1 ("cas faux"), "Plot.Point Style"=i8 9 ("cas faux"), "Plot.Visible?"=TRUE, "Plot.Fill/Pt. Color"=w328) -> (error out=w327:errorcluster)  [unwired: 2 in, 1 out]
              }
              n199 = for {
                tunnel: w315 -> [w326] mode=indexing
                tunnel: w313 -> [w325] mode=indexing
                tunnel: [w324] -> w314 mode=indexing
                n200 = Bundle By Name(cluster=w326, "couleur"=w325, "Y1"=FALSE, "Y2"=TRUE) -> (w324:T8)
              }
              n201 = local write "Légende"(w314) -> ()
              n202 = property on="Courbe" class="GraphXY (strict)"(error in=w317, "ActYScl"=0 ("Échelle active des Y"), "YScale.Visible"=FALSE ("Échelle des Y.Visible"), "ActYScl"=1 ("Échelle active des Y"), "YScale.Visible"=TRUE ("Échelle des Y.Visible")) -> (error out=w316:errorcluster)  [unwired: 1 in, 1 out]
              n203 = call <vilib>:"Clear Errors.vi"("error in (no error)"=w316) -> ()  [unwired: 5 in, 2 out]
            }
            event "Tout OFF": Value Change {
              n204 = event-data() -> ()  [unwired: 1 in, 5 out]
              n205 = local read "Légende"() -> (w334:T1)
              n206 = for {
                tunnel: [w345] -> w336
                tunnel: w334 -> [w344] mode=indexing
                tunnel: [w342] -> w333 mode=indexing
                i -> [w346]
                w341 = FALSE ("Y1")
                n207 = property on="Courbe" class="GraphXY (strict)"("Active Plot"=w346, "Plot.Visible?"=FALSE) -> (error out=w345:errorcluster)  [unwired: 2 in, 1 out]
                n208 = Bundle By Name(cluster=w344, "couleur"=u32 16777216 ("nouvel élément/sous-tableau"), "Y1"=w341, "Y2"=w341) -> (w342:T8)
              }
              n209 = local write "Légende"(w333) -> ()
              n210 = property on="Courbe" class="GraphXY (strict)"(error in=w336, "ActYScl"=0 ("Échelle active des Y"), "YScale.Visible"=FALSE ("Échelle des Y.Visible"), "ActYScl"=1 ("Échelle active des Y"), "YScale.Visible"=FALSE ("Échelle des Y.Visible")) -> (error out=w335:errorcluster)  [unwired: 1 in, 1 out]
              n211 = call <vilib>:"Clear Errors.vi"("error in (no error)"=w335) -> ()  [unwired: 5 in, 2 out]
            }
            event "Calcul Pente": Value Change {
              n212 = event-data() -> ("NewVal"=w348:bool)  [unwired: 1 in, 5 out]
              n213 = property on="Courbe" class="GraphXY (strict)"() -> ("XScale.Maximum"=w356:dbl, "XScale.Minimum"=w352:dbl)  [unwired: 2 in, 2 out]
              n214 = property on="Pente" class="NumNb (strict)"("Visible"=w348) -> ()  [unwired: 2 in, 2 out]
              n215 = property on="Unités par" class="MDér (strict)"("Visible"=w348) -> ()  [unwired: 2 in, 2 out]
              n216 = property on="Capteur" class="MDér (strict)"("Visible"=w348) -> ()  [unwired: 2 in, 2 out]
              n217 = property on="Courbe" class="GraphXY (strict)"("Active Cursor"=u32 0 ("Curseur actif"), "Cursor.Visible"=w348, "Active Cursor"=u32 1 ("Curseur actif"), "Cursor.Visible"=w348) -> ()  [unwired: 2 in, 2 out]
              n218 = Subtract(x=w356, y=w352) -> (x-y=w355:dbl)
              n219 = Divide(x=w355, y=2.0) -> (x/y=w353:dbl)
              n220 = Add(x=w353, y=w352) -> (x+y=w351:dbl)
              n221 = property on="Courbe" class="GraphXY (strict)"("Active Cursor"=u32 0 ("Curseur actif"), "Cursor.Cursor X"=w351, "Active Cursor"=u32 1 ("Curseur actif"), "Cursor.Cursor X"=w351) -> ()  [unwired: 2 in, 2 out]
            }
            event "Unités par", "Capteur": Value Change; "Courbe": Cursor Release {
              n222 = event-data() -> ()  [unwired: 1 in, 4 out]
              n223 = property on="Courbe" class="GraphXY (strict)"("Active Cursor"=u32 0 ("Curseur actif"), "Cursor.Cursor Plot"="Capteur", "Active Cursor"=u32 1 ("Curseur actif"), "Cursor.Cursor Plot"="Capteur") -> ("Cursor.Cursor X"=w360:dbl, "Cursor.Cursor Y"=w361:dbl, "Cursor.Cursor X"=w362:dbl, "Cursor.Cursor Y"=w363:dbl)  [unwired: 2 in, 2 out]
              n224 = Max & Min(x=w361, y=w363) -> (max(x,y)=w372:dbl, min(x,y)=w371:dbl)
              n225 = Max & Min(x=w360, y=w362) -> (max(x,y)=w370:dbl, min(x,y)=w369:dbl)
              n226 = Subtract(x=w372, y=w371) -> (x-y=w368:dbl)
              n227 = Subtract(x=w370, y=w369) -> (x-y=w367:dbl)
              n228 = Divide(x=w368, y=w367) -> (x/y=w366:dbl)
              n229 = case shown="1" "Unités par" {
                tunnel: w366 -> [w375 w376 w380]
                tunnel: [w375 w377 w379] -> w365
                frame 0, Default {
                  # "seconde"
                }
                frame 1 {
                  # "minute"
                  n230 = Multiply(x=w376, y=60.0) -> (x*y=w377:dbl)
                }
                frame 2 {
                  # "heure"
                  n231 = Multiply(x=w380, y=3600.0) -> (x*y=w379:dbl)
                }
              }
              "Pente" <- w365
            }
            event "SORTIR VISU": Value Change {
              n232 = event-data() -> ("NewVal"=w382:bool)  [unwired: 1 in, 4 out]
              n233 = case shown="Vrai" w382 {
                frame False {
                }
                frame True {
                  n234 = call "Boite Dialogue 2 boutons.vi"("bouton droit visible ?"=TRUE, "Texte bouton droit"="OUI" ("Texte bouton gauche"), "Texte bouton gauche"="NON" ("Texte bouton droit"), "Message"="Vous avez demandé de sortir de la visualisation graphique.\nA la prochaine ouverture, le graphe sera réinitialisé\n(il ne comportera que le dernier fichier)\nVoulez-vous continuer ?") -> ("Bouton droit ?"=→"SORTIE VISU":bool)
                  n235 = local write "SORTIR VISU"(FALSE ("SORTIR VISU")) -> ()
                }
              }
            }
          }
          n236 = global read "Variable glob generale.vi" "Lancement"() -> (w162:bool)
          n237 = local read "SORTIE VISU"() -> (w163:bool)
          n238 = Not(x=w162) -> (.not. x?=w161:bool)
          n239 = Or(x=w163, y=w161) -> (x .or. y?=w164:bool)
        }
        n240 = Not Equal?(x=w158, y="") -> (x != y?=w156:bool)
        n241 = local read "nb capt"() -> (w154:i32)
        n242 = property on="commentaire" class="Ch"("Visible"=w156) -> ()  [unwired: 2 in, 2 out]
        n243 = while {
          shift-right: [w406] -> _
          shift-left: w160 -> [w408]
          shift-right: [w405] -> _
          shift-left: w159 -> [w407]
          shift-right: [w404] -> _
          shift-left: _ -> [w403]
          tunnel: w154 -> [w402]
          tunnel: w155 -> [w390]
          stop <- w394 stop-if-true
          # "données"
          # "temps"
          n244 = feedback #1(w390) -> (w391:i64)
          n245 = call "Nouvelles donnees.vi"("Nb Capteurs"=w402, "offset entrée (en octets) (0)"=w391) -> ("Nouvelles données"=w389:string[], "Nouveau temps"=w404:dbl, "Chemin du fichier local :"=→"Chemin du fichier local":path, "offset sortie (en octets)"=w392:i64)
          n246 = feedback-in #1(w392) -> ()
          n247 = Equal?(x=w403, y=w404) -> (x = y?=w400:bool)
          n248 = Equal To 0?(x=w404) -> (x = 0?=w399:bool)
          n249 = Or(x=w400, y=w399) -> (x .or. y?=w398:bool)
          n250 = case shown="Faux" w398 {
            tunnel: w408 -> [w422 w449]
            tunnel: w407 -> [w429 w448]
            tunnel: [w433 w449] -> w406
            tunnel: [w426 w448] -> w405
            tunnel: w389 -> [w424 _]
            tunnel: w404 -> [w428 _]
            frame False {
              # "12h pour 28 capteurs\ntoutes les 1s"
              n251 = Array Size(array=w422) -> (size(s)=w421:i32[])
              n252 = Index Array(array=w421, index #1=0 ("indice"), index #2=1 ("indice")) -> (element #1=w417:i32, element #2=w418:i32)
              n253 = Multiply(x=w417, y=w418) -> (x*y=w416:i32)
              n254 = Fract/Exp String To Number(string=w424) -> (number=w425:dbl[])  [unwired: 3 in, 1 out]
              n255 = Greater?(x=w416, y=1200000) -> (0:w423:bool)
              n256 = case shown="Vrai" w423 {
                tunnel: [w434 w436] -> w431
                tunnel: [w435 w437] -> w430
                tunnel: w429 -> [w434 w443]
                tunnel: w422 -> [w435 w440]
                frame False {
                }
                frame True {
                  n257 = Delete From Array(array=w443, length=1 ("longueur"), index=0 ("indice")) -> (array with subset deleted=w436:dbl[])  [unwired: 1 out]
                  n258 = Delete From Array(array=w440, length=1 ("longueur"), index (row)=0 ("indice (ligne)")) -> (array with subset deleted=w437:dbl[][])  [unwired: 1 in, 1 out]
                }
              }
              n259 = Build Array (concatenate)(w430, w425) -> (w433:dbl[][])
              n260 = Build Array (concatenate)(w431, w428) -> (w426:dbl[])
              n261 = Transpose 2D Array(2D array=w433) -> (transposed array=w427:dbl[][])
              n262 = for {
                tunnel: w427 -> [w445] mode=indexing
                tunnel: w426 -> [w446]
                tunnel: [w447] -> w432 mode=indexing
                n263 = Bundle(w446, w445) -> (w447:cluster{dbl[], dbl[]})  [unwired: 1 in]
                n264 = Wait (ms)(milliseconds to wait=u32 10 ("attente (ms)")) -> ()  [unwired: 1 out]
              }
              "Courbe" <- w432
            }
            frame True {
              # "pas de nouvelles données\nou ligne vide => temps = 0"
            }
          }
          n265 = Wait Until Next ms Multiple(millisecond multiple=u32 1000 ("n millisecondes")) -> ()  [unwired: 1 out]
          n266 = flat-sequence {
            tunnel: w389 -> [w410]
            frame #0 {
              n267 = local read "Légende"() -> (w409:T1)
              n268 = for {
                tunnel: w409 -> [w414] mode=indexing
                tunnel: [w413] -> w411 mode=indexing
                tunnel: w410 -> [w412] mode=indexing
                n269 = Bundle By Name(cluster=w414, "donnée"=w412) -> (w413:T8)
              }
              n270 = local write "Légende"(w411) -> ()
            }
          }
          n271 = local read "SORTIE VISU"() -> (w396:bool)
          n272 = global read "Variable glob generale.vi" "Lancement"() -> (w395:bool)
          n273 = Not(x=w395) -> (.not. x?=w393:bool)
          n274 = Or(x=w396, y=w393) -> (x .or. y?=w394:bool)
        }
      }
      frame "fin" {
        # "enregistrement des couleurs"
        n275 = global read "Variable glob generale.vi" "Couleurs"() -> (w450:u32[])
        n276 = disable-structure shown="Activé" {
          disable-tunnel: [w468 w476] -> w457
          disable-tunnel: w450 -> [w467 w477]
          frame Disabled {
            n277 = Array To Spreadsheet String(delimiter (Tab)=";" ("séparateur (Tabulation)"), array=w467, 3:"%d" ("chaîne de format")) -> (spreadsheet string=w469:string)
            n278 = String Length(string=w469) -> (length=w473:i32)
            n279 = Subtract(x=w473, y=2) -> (x-y=w471:i32)
            n280 = String Subset(string=w469, offset (0)=0, length (rest)=w471) -> (substring=w468:string)
          }
          frame Enabled {
            n281 = Number To Fractional String(number=w477, precision (6)=i16 2 ("précision (6)")) -> (F-format string=w479:string[])  [unwired: 2 in]
            n282 = call "Tableau en chaine.vi"("Tableau 1D"=w479) -> ("Chaîne"=w476:string)  [unwired: 1 in, 1 out]
          }
        }
        n283 = disable-structure shown="Activé" {
          frame Enabled {
            n284 = local read "référence en sortie"() -> (w483:refnum<vi>)
            n285 = invoke class="VI" method="FA.Fermer"(reference=w483) -> (reference out=w481:refnum<vi>, error out=w482:errorcluster)  [unwired: 2 in, 1 out]
            n286 = Close Reference(reference=w481, error in (no error)=w482) -> (error out=w480:errorcluster)
            n287 = call <vilib>:"Clear Errors.vi"("error in (no error)"=w480) -> ()  [unwired: 5 in, 2 out]
          }
          frame Disabled {
          }
        }
        n288 = Request Deallocation(TRUE ("flag")) -> ()
        n289 = Build Path(base path=path "C:/LABVIEW/PRES+TEMP+REG dernière version/Configurations", name or relative path="config acqui.ini" ("nom ou chemin relatif")) -> (appended path=w465:path)
        n290 = call <vilib>:"Open Config Data.vi"("create file if necessary (T)"=TRUE ("create file if necessary? (T)"), "configuration file path"=w465) -> ("error out"=w463:errorcluster, "refnum"=w462:T14)  [unwired: 7 in, 1 out]
        n291 = call-poly <vilib>:"Write Key.vi"("section"="GENERAL", "error in (no error)"=w463, "value"=w457, "key"="COULEURS", "refnum"=w462) -> ("error out"=w458:errorcluster, "refnum out"=w459:T14)  [unwired: 4 in, 1 out]
        n292 = call <vilib>:"Close Config Data.vi"("error in (no error)"=w458, "refnum"=w459) -> ("error out"=w455:errorcluster)  [unwired: 8 in, 1 out]
        n293 = call <vilib>:"Clear Errors.vi"("error in (no error)"=w455) -> ()  [unwired: 5 in, 2 out]
        n294 = global write "Variable glob generale.vi" "Visu en cours"(FALSE ("Visu en cours")) -> ()
      }
    }
  }
